vi "Populate gRPC Events.vi"(7 "RPC Method Parameters":T1[](array[typedef]), 8 "error in (no error)":errorcluster, 11 "Server class in":refnum<vi>) -> (0 "error out":errorcluster, 3 "Server class out":refnum<vi>)   [LabVIEW 2019, in "gRPC Template Creation Utility.lvlib"]
uses:
  gRPC Template Creation Utility.lvlib
  TypeDefs/RPC Method Parameters.ctl
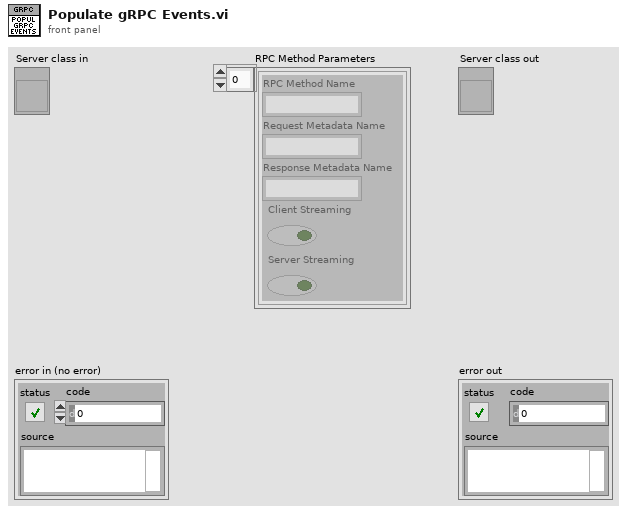
[diagram p1: front panel]
types:
  T1 = typedef "gRPC Template Creation Utility.lvlib/RPC Method Parameters.ctl" = cluster{"RPC Method Name":string, "Request Metadata Name":string, "Response Metadata Name":string, "Client Streaming":bool, "Server Streaming":bool}
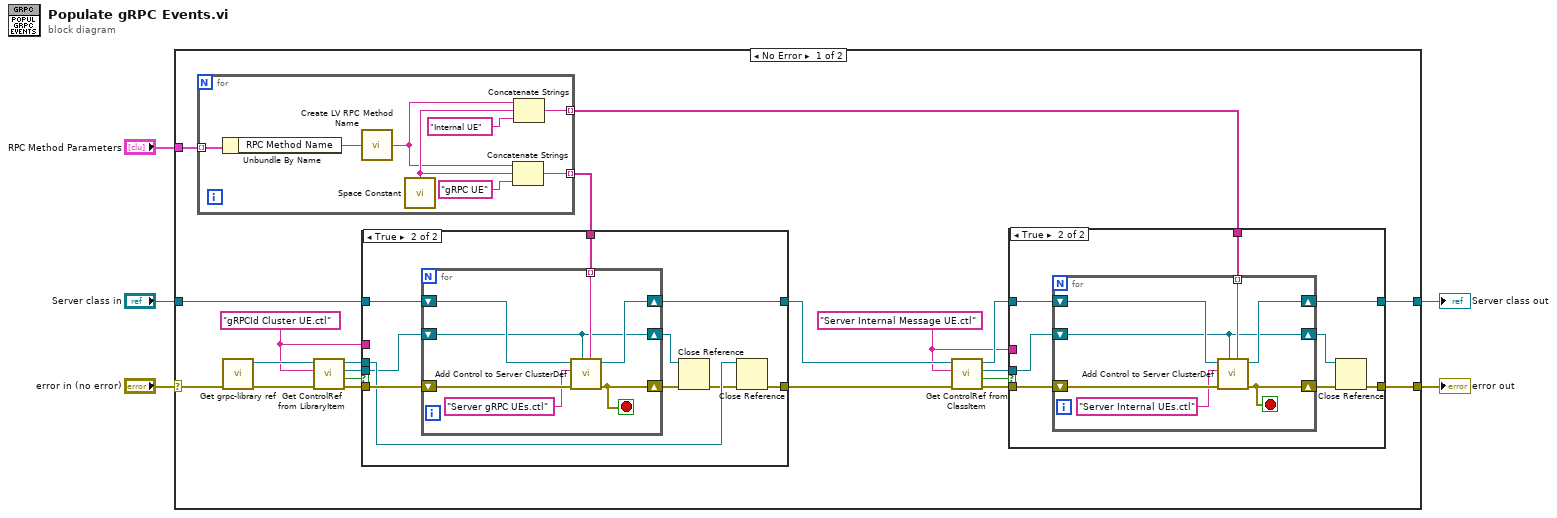
[diagram p0: block diagram]
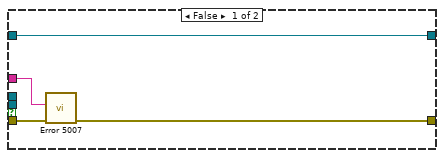
[diagram p2: hidden frame]
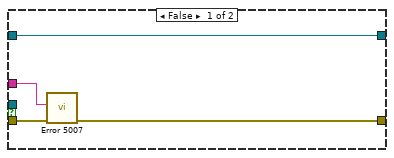
[diagram p3: hidden frame]
diagram:
  n1 = case shown="No Error" "error in (no error)" {
    selector: "error in (no error)" -> [w15 w75]
    tunnel: [w11 w75] -> w5
    tunnel: [w26 w76] -> w4
    tunnel: "Server class in" -> [w6 w76]
    tunnel: "RPC Method Parameters" -> [w14 _]
    frame No Error {
      w9 = "Server Internal Message UE.ctl" ("Item Name")
      w7 = "gRPCId Cluster UE.ctl" ("y")
      n2 = for {
        tunnel: w14 -> [w74] mode=indexing
        tunnel: [w72] -> w13 mode=indexing
        tunnel: [w70] -> w12 mode=indexing
        n3 = Unbundle By Name(w74) -> ("RPC Method Name"=w68:string)
        n4 = call "Create LV RPC Method Name.vi"("Proto Parser RPC Method Name in"=w68) -> ("LV RPC Method Name out"=w67:string)
        n5 = call <vilib>:"Space Constant.vi"() -> ("String"=w69:string)
        n6 = Concatenate Strings(w67, w69, "gRPC UE" ("string")) -> (w72:string)
        n7 = Concatenate Strings(w67, w69, "Internal UE" ("string")) -> (w70:string)
      }
      n8 = call "Get grpc-library ref.vi"("error in"=w15) -> ("error out"=w17:errorcluster, "Library out"=w16:refnum<vi>)  [unwired: 9 in]
      n9 = call "Get ControlRef from LibraryItem.vi"("error in (no error)"=w17, "Control Name"=w7, "Library item in"=w16) -> ("error out"=w24:errorcluster, "Found?"=w8:bool, "Control ref out"=w22:refnum<vi>, "Library item out"=w23:refnum<vi>)  [unwired: 5 in]
      n10 = case shown="True" w8 {
        tunnel: [w27 w40] -> w25
        tunnel: w6 -> [w30 w39]
        tunnel: w24 -> [w29 w38]
        tunnel: w23 -> [_ w37]
        tunnel: w22 -> [_ w35]
        tunnel: [w30 w33] -> w18
        tunnel: w13 -> [_ w32]
        tunnel: w7 -> [w28 _]
        frame False {
          n11 = call "Error 5007.vi"("error in (no error)"=w29, "Target ClusterDef Name"=w28) -> ("error out"=w27:errorcluster)  [unwired: 9 in]
        }
        frame True {
          n12 = for {
            shift-right: [w43] -> w34
            shift-left: w38 -> [w47]
            tunnel: w32 -> [w45] mode=indexing
            shift-right: [w44] -> w33
            shift-left: w39 -> [w46]
            shift-right: [w41] -> w31
            shift-left: w35 -> [w41]
            stop <- w43 stop-if-true
            n13 = call "Add Control to Server ClusterDef.vi"("New Control Label"=w45, "Source Control ref in"=w41, "error in (no error)"=w47, "Target ClusterDef Name"="Server gRPC UEs.ctl" ("Item Name"), "Server class in"=w46) -> ("error out"=w43:errorcluster, "Server class out"=w44:refnum<vi>)  [unwired: 5 in]
          }
          n14 = Close Reference(reference=w31, error in (no error)=w34) -> (error out=w36:errorcluster)
          n15 = Close Reference(reference=w37, error in (no error)=w36) -> (error out=w40:errorcluster)
        }
      }
      n16 = call "Get ControlRef from ClassItem.vi"("error in (no error)"=w25, "Item Name"=w9, "LVClassLibrary in"=w18) -> ("error out"=w20:errorcluster, "Found ?"=w10:bool, "Control ref out"=w21:refnum<vi>, "LVClassLibrary out"=w19:refnum<vi>)  [unwired: 5 in]
      n17 = case shown="True" w10 {
        tunnel: [w51 w59] -> w26
        tunnel: w21 -> [_ w58]
        tunnel: w20 -> [w50 w57]
        tunnel: w19 -> [w51 w56]
        tunnel: w12 -> [_ w55]
        tunnel: [w49 w52] -> w11
        tunnel: w9 -> [w48 _]
        frame False {
          n18 = call "Error 5007.vi"("error in (no error)"=w50, "Target ClusterDef Name"=w48) -> ("error out"=w49:errorcluster)  [unwired: 9 in]
        }
        frame True {
          n19 = for {
            tunnel: w55 -> [w64] mode=indexing
            shift-right: [w63] -> w59
            shift-left: w56 -> [w65]
            shift-right: [w62] -> w54
            shift-left: w57 -> [w66]
            shift-right: [w61] -> w53
            shift-left: w58 -> [w61]
            stop <- w62 stop-if-true
            n20 = call "Add Control to Server ClusterDef.vi"("New Control Label"=w64, "Source Control ref in"=w61, "error in (no error)"=w66, "Target ClusterDef Name"="Server Internal UEs.ctl", "Server class in"=w65) -> ("error out"=w62:errorcluster, "Server class out"=w63:refnum<vi>)  [unwired: 5 in]
          }
          n21 = Close Reference(reference=w53, error in (no error)=w54) -> (error out=w52:errorcluster)
        }
      }
    }
    frame Error {
    }
  }
  "error out" <- w5
  "Server class out" <- w4
